vi "Test CAN Status.vi"() -> ()   [LabVIEW 2021]
uses:
  CAN RW CANsub.lvclass
  <vilib>/CIF Foundation/CIF CAN RW Core/CAN_RW_CORE.lvclass
  <vilib>/CIF Foundation/CIF PCAP Parse and Build/pcap_Parse_Build_CIF.lvclass
  <vilib>/CIF Foundation/CIF PCAP Parse and Build/Typedef/Format Specific/CAN Interface Mode.ctl
  <vilib>/CIF Foundation/CIF PCAP Parse and Build/Typedef/Format Specific/CAN Metadata.ctl
  <vilib>/CIF Foundation/CIF CAN RW Core/typedef/Communication State.ctl
  <vilib>/CIF Foundation/CIF CAN RW Core/typedef/Last Error.ctl
  <vilib>/CIF Foundation/CIF CAN RW Core/typedef/CAN Status.ctl
panel:
  in  "wait between calls ms":u32
  out "error out":errorcluster
  out "call time ms":dbl[](array[numeric])
  out "CAN Status":T1
  in  "send one frame":bool
  in  "Interface":string="192.168.0.49/1"
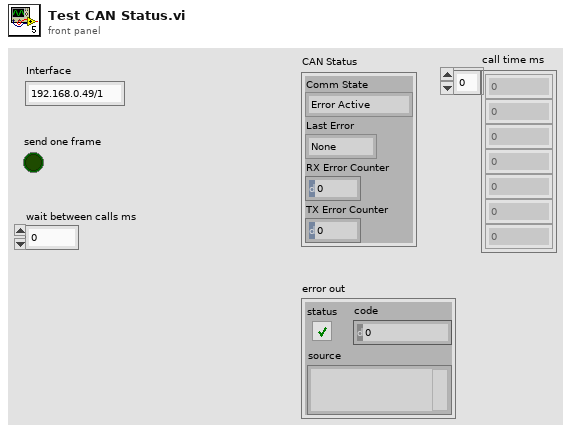
[diagram p1: front panel]
types:
  T1 = typedef "CAN_RW_CORE.lvclass/CAN Status.ctl" = cluster{"Comm State":T2, "Last Error":T3, "RX Error Counter":u8, "TX Error Counter":u8}
  T2 = typedef "CAN_RW_CORE.lvclass/Communication State.ctl" = enum16{"Error Active", "Error Passive", "Bus Off"}
  T3 = typedef "CAN_RW_CORE.lvclass/Last Error.ctl" = enum16{"None", "Stuff", "Form", "Ack", "Bit1", "Bit0", "CRC", "Unknown"}
  T4 = typedef "pcap_Parse_Build_CIF.lvclass/CAN Interface Mode.ctl" = enum16{"CAN 2.0", "CAN FD", "CAN FD BRS", "Remote"}
  T5 = typedef "pcap_Parse_Build_CIF.lvclass/CAN Metadata.ctl" = cluster{"TAI Time (ns)":i64, "identifier":u32, "extended?":bool, "Interface Mode":T4}
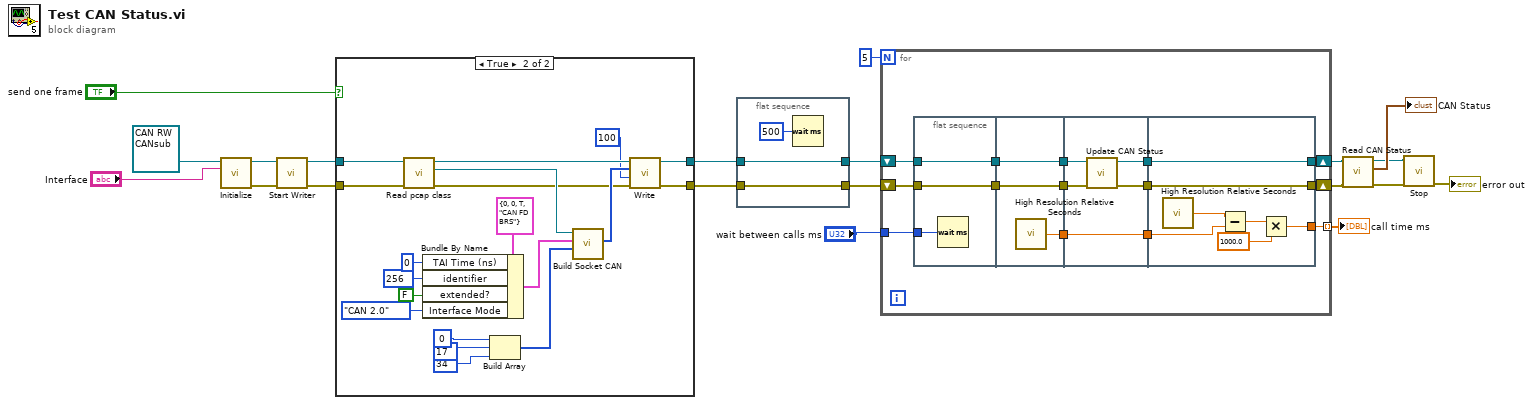
[diagram p0: block diagram]
diagram:
  n1 = call "Initialize.vi"("Interface"="Interface", "CANsub_CAN_RW in"=refnum<class "CAN RW CANsub.lvclass"> refnum ("CAN RW CANsub.lvclass")) -> ("error out"=w17:errorcluster, "CANsub_CAN_RW out"=w18:refnum<class "CAN RW CANsub.lvclass">)  [unwired: 8 in]
  n2 = call-dynamic "Start Writer.vi"("error in (no error)"=w17, "CAN RW CANsub in"=w18) -> ("error out"=w14:errorcluster, "CAN RW CANsub out"=w15:refnum<class "CAN RW CANsub.lvclass">)  [unwired: 8 in]
  n3 = case shown="True" "send one frame" {
    tunnel: [w22 w24] -> w13
    tunnel: w15 -> [w22 w41]
    tunnel: [w21 w23] -> w12
    tunnel: w14 -> [w21 w40]
    frame False {
    }
    frame True {
      n4 = call <vilib>:"Read pcap class.vi"("error in (no error)"=w40, "CAN_RW_CORE in"=w41) -> ("error out"=w26:errorcluster, "pcap class"=w38:refnum<class "pcap_Parse_Build_CIF.lvclass">, "CAN_RW_CORE out"=w28:refnum<class "CAN RW CANsub.lvclass">)  [unwired: 7 in]
      n5 = Bundle By Name(cluster=T5 {"TAI Time (ns)"=0, "identifier"=0, "extended?"=TRUE, "Interface Mode"=enum."CAN FD BRS"} ("CAN Metadata"), "TAI Time (ns)"=i64 0, "identifier"=u32 256, "extended?"=FALSE, "Interface Mode"=CAN_Interface_Mode."CAN 2.0") -> (w37:T5)
      n6 = Build Array(u8 0, u8 17, u8 34) -> (w29:u8[])
      n7 = call <vilib>:"Build Socket CAN.vi"("Payload"=w29, "CAN Metadata"=w37, "pcap Parse and Build in"=w38) -> ("CAN Packet"=w27:u8[])  [unwired: 7 in, 1 out]
      n8 = call-dynamic "Write.vi"("error in (no error)"=w26, "timeout (ms)"=100, "pcap CAN DATA in"=w27, "CAN RW CANsub in"=w28) -> ("error out"=w23:errorcluster, "CAN RW CANsub out"=w24:refnum<class "CAN RW CANsub.lvclass">)  [unwired: 5 in, 1 out]
    }
  }
  n9 = flat-sequence {
    tunnel: [w44] -> w10
    tunnel: w13 -> [w44]
    tunnel: [w43] -> w9
    tunnel: w12 -> [w43]
    frame #0 {
      n10 = Wait (ms)(milliseconds to wait=u32 500) -> ()  [unwired: 1 out]
    }
  }
  n11 = for {
    N: 5 -> [_]
    shift-right: [w54] -> w7
    shift-left: w10 -> [w57]
    shift-right: [w52] -> w6
    shift-left: w9 -> [w55]
    tunnel: [w48] -> w8 mode=indexing
    tunnel: "wait between calls ms" -> [w45]
    n12 = flat-sequence {
      tunnel: w55 -> [w60]
      tunnel: w57 -> [w61]
      tunnel: [w61] -> w47
      tunnel: [w60] -> w46
      tunnel: w45 -> [w59]
      tunnel: [w64] -> w58
      tunnel: [w63] -> w56
      tunnel: [w62] -> w49
      tunnel: w47 -> [w64]
      tunnel: w46 -> [w63]
      tunnel: w58 -> [w69]
      tunnel: w56 -> [w68]
      tunnel: [w67] -> w53
      tunnel: [w66] -> w51
      tunnel: [w65] -> w50
      tunnel: w49 -> [w65]
      tunnel: [w76] -> w54
      tunnel: w53 -> [w76]
      tunnel: [w75] -> w52
      tunnel: w51 -> [w75]
      tunnel: w50 -> [w73]
      tunnel: [w71] -> w48
      frame #0 {
        n13 = Wait (ms)(milliseconds to wait=w59) -> ()  [unwired: 1 out]
      }
      frame #1 {
        n14 = call <vilib>:"High Resolution Relative Seconds.vi"() -> ("relative seconds"=w62:dbl)
      }
      frame #2 {
        n15 = call "Update CAN Status.vi"("error in (no error)"=w68, "CAN RW CANsub in"=w69) -> ("error out"=w66:errorcluster, "CAN RW CANsub out"=w67:refnum<class "CAN RW CANsub.lvclass">)  [unwired: 8 in]
      }
      frame #3 {
        n16 = call <vilib>:"High Resolution Relative Seconds.vi"() -> ("relative seconds"=w74:dbl)
        n17 = Subtract(x=w74, y=w73) -> (x-y=w72:dbl)
        n18 = Multiply(x=w72, y=1000.0) -> (x*y=w71:dbl)
      }
    }
  }
  "call time ms" <- w8
  n19 = call <vilib>:"Read CAN Status.vi"("error in (no error)"=w6, "CAN_RW_CORE in"=w7) -> ("error out"=w3:errorcluster, "CAN Status"=→"CAN Status":T1, "CAN_RW_CORE out"=w4:refnum<class "CAN RW CANsub.lvclass">)  [unwired: 7 in]
  n20 = call-dynamic "Stop.vi"("error in (no error)"=w3, "CAN RW CANsub in"=w4) -> ("error out"=→"error out":errorcluster)  [unwired: 8 in, 1 out]
